vi "PicoScope6000aSetupStreaming.vi"(0 "handle in":i16=16384, 1 "Streaming Acquisition Settings":T5={"preTriggerSamples"=0, "postTriggerSamples"=1000000, "Requested sampleInterval"=1.0, "sampleIntervalTimeUnits"=3} {"sampleIntervalTimeUnits" items=["femtoseconds", "picoseconds", "nanoseconds", "microseconds", "millseconds", "seconds"]; "postTriggerSamples" format="%_6p"; "preTriggerSamples" format="%_6p"}, 2 "Buffer and Transfer Settings":T4={"startIndex"=0, "Samples"=1000000, "Down Sample Ratio"=1, "Down-Sample Mode"=2147483648} {"Down-Sample Mode" items=["None"=2147483648, "Aggregate"=1, "Decimate"=2, "Average"=4]; "Down Sample Ratio" step=1; "Samples" format="%_6p"}, 3 "enabled array":i16[](array[numeric])=[1, 1, 0, 0, 0, 0, 0, 0, 0, 0], 5 "Device Info":T1, 7 "Data Pointers In":T2, 9 "Number of Buffers":i32=1, 11 "error in (no error)":errorcluster, 12 "Auto Stop":bool) -> (4 "handle out":i16=16384, 8 "Data Pointers":T2, 13 "Actual sampleInterval":T3, 15 "error out":errorcluster)   [LabVIEW 2016]
doc: "Setup streaming Pico data buffers and first calls to ps6000aSetDataDataBuffer"
uses:
  ps6000a.dll
  shared/PicoBuffers.ctl
panel:
  in  "Dummy enabled array":i16[](array[numeric])=[1, 1, 1, 1, 1, 1, 1, 1, 1, 1]
  out "Actionflag":bool=TRUE
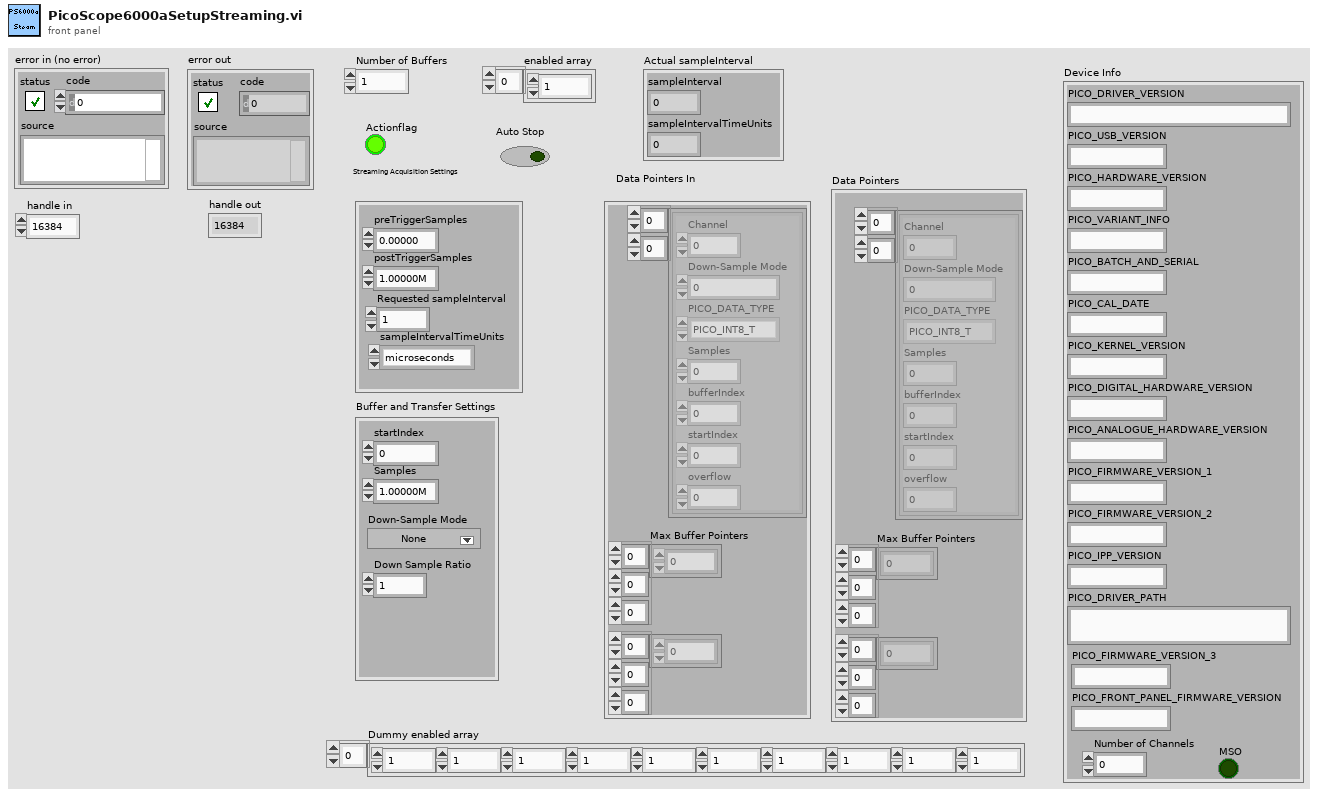
[diagram p1: front panel]
types:
  T1 = cluster{"PICO_DRIVER_VERSION":string, "PICO_USB_VERSION":string, "PICO_HARDWARE_VERSION":string, "PICO_VARIANT_INFO":string, "PICO_BATCH_AND_SERIAL":string, "PICO_CAL_DATE":string, "PICO_KERNEL_VERSION":string, "PICO_DIGITAL_HARDWARE_VERSION":string, "PICO_ANALOGUE_HARDWARE_VERSION":string, "PICO_FIRMWARE_VERSION_1":string, "PICO_FIRMWARE_VERSION_2":string, "PICO_IPP_VERSION":string, "PICO_DRIVER_PATH":string, "PICO_FIRMWARE_VERSION_3":string, "PICO_FRONT_PANEL_FIRMWARE_VERSION":string, "Number of Channels":i16, "MSO":bool}
  T2 = typedef "PicoBuffers.ctl" = cluster{"Max Buffer Pointers":u64[][][], "Min Buffer Pointers":u64[][][], "StreamingDataInfo":cluster{"Channel":u32, "Down-Sample Mode":u32, "PICO_DATA_TYPE":enum32{"PICO_INT8_T", "PICO_INT16_T", "PICO_INT32_T", "PICO_UINT32_T", "PICO_INT64_T", ""}, "Samples":i32, "bufferIndex":u64, "startIndex":i32, "overflow":i16}[][]}
  T3 = cluster{"sampleInterval":dbl, "sampleIntervalTimeUnits":u32}
  T4 = cluster{"startIndex":u64, "Samples":u64, "Down Sample Ratio":u64, "Down-Sample Mode":u32}
  T5 = cluster{"preTriggerSamples":u64, "postTriggerSamples":u64, "Requested sampleInterval":dbl, "sampleIntervalTimeUnits":u32}
  T6 = enum32{"PICO_INT8_T", "PICO_INT16_T", "PICO_INT32_T", "PICO_UINT32_T", "PICO_INT64_T", ""}
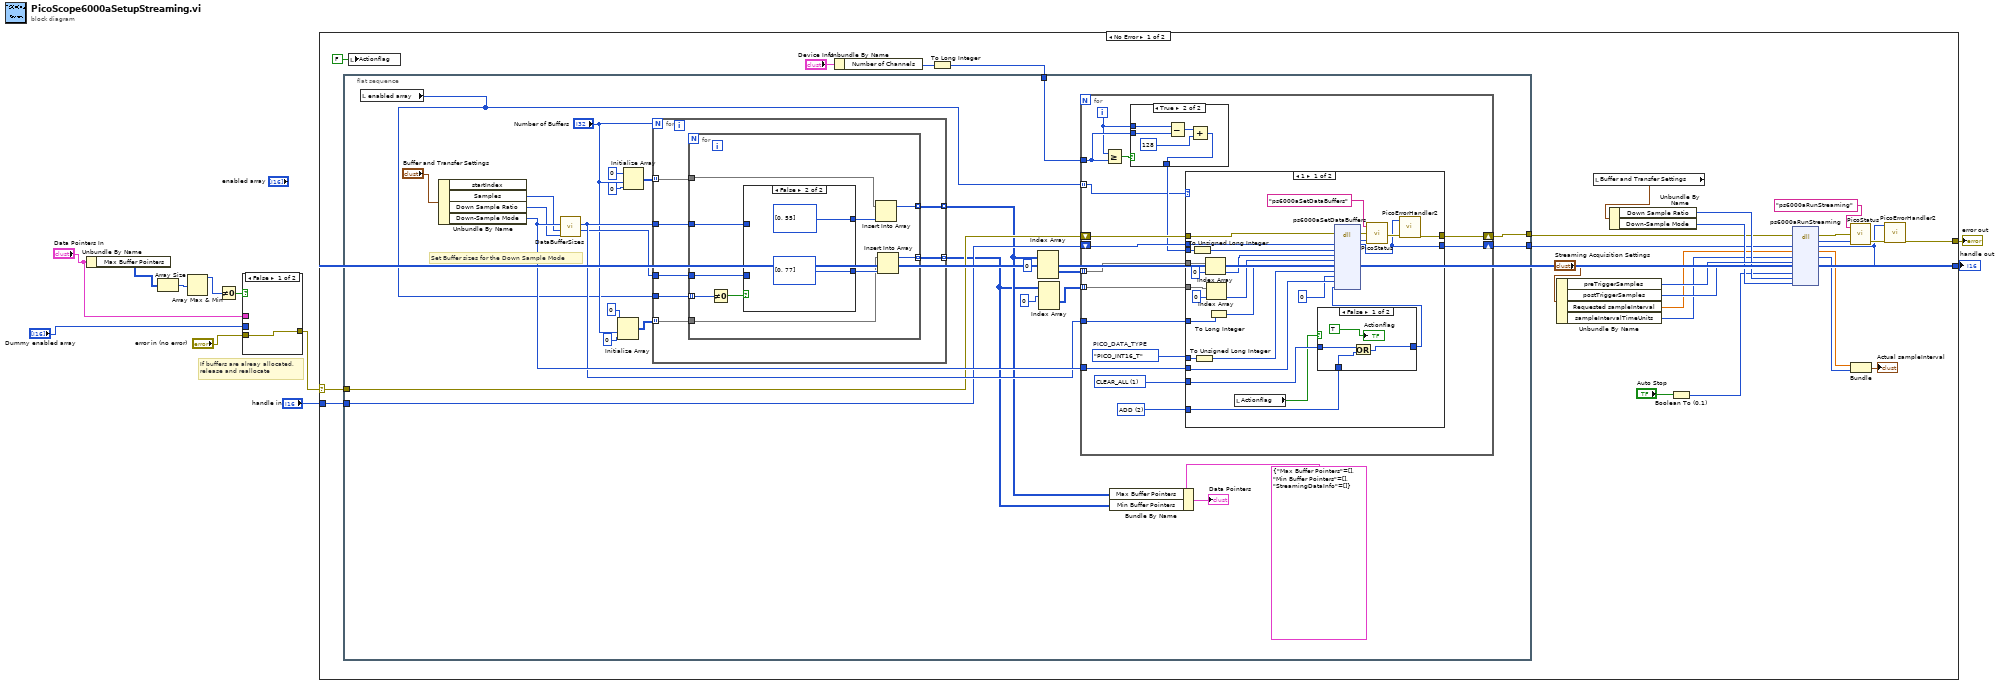
[diagram p0: block diagram]
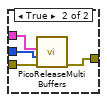
[diagram p2: hidden frame]
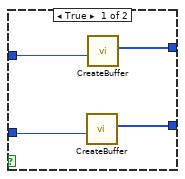
[diagram p6: hidden frame]
diagram:
  # "If buffers are alreay allocated,\nrelease and reallocate"
  n1 = Unbundle By Name("Data Pointers In") -> ("Max Buffer Pointers"=w3:u64[][][])
  n2 = Array Size(array=w3) -> (size(s)=w7:i32[])
  n3 = Array Max & Min(array=w7) -> (max value=w6:i32)  [unwired: 3 out]
  n4 = Not Equal To 0?(x=w6) -> (x != 0?=w8:bool)
  n5 = case shown="False" w8 {
    tunnel: "error in (no error)" -> [w12 w16]
    tunnel: [w12 w15] -> w4
    tunnel: "Dummy enabled array" -> [_ w14]
    tunnel: "Data Pointers In" -> [_ w13]
    frame False {
    }
    frame True {
      n6 = call "PicoReleaseMultiBuffers.vi"("error in (no error)"=w16, "Enabled array"=w14, "Data Pointers"=w13) -> ("error out"=w15:errorcluster)  [unwired: 8 in]
    }
  }
  n7 = case shown="No Error" w4 {
    selector: w4 -> [w33 w149]
    tunnel: "handle in" -> [w32 w150]
    tunnel: [w25 w150] -> w10
    tunnel: [w26 w149] -> w9
    frame No Error {
      n8 = flat-sequence {
        tunnel: w33 -> [w53]
        tunnel: w32 -> [w54]
        tunnel: [w55] -> w31
        tunnel: [w50] -> w30
        tunnel: w18 -> [w44]
        frame #0 {
          # "Set Buffer sizes for the Down Sample Mode"
          n9 = local read "enabled array"() -> (w45:i16[])
          n10 = Unbundle By Name("Buffer and Transfer Settings") -> ("Samples"=w63:u64, "Down Sample Ratio"=w62:u64, "Down-Sample Mode"=w64:u32)  [unwired: 1 out]
          n11 = call "DataBufferSizes.vi"("Down Sample Ratio"=w62, "Number of Samples"=w63, "Down-Sample Mode"=w64) -> ("min Buffer Size"=w60:i32, "Max Buffer Size"=w61:i32)  [unwired: 7 in]
          n12 = Initialize Array(u64 0 ("element"), "Number of Buffers", 0 ("dimension size")) -> (w57:u64[][])
          n13 = Initialize Array(u64 0 ("element"), "Number of Buffers", 0 ("dimension size")) -> (w65:u64[][])
          n14 = for {
            N: "Number of Buffers" -> [_]
            tunnel: w45 -> [w131]
            tunnel: w61 -> [w132]
            tunnel: w60 -> [w130]
            tunnel: [w129] -> w49 mode=indexing
            tunnel: w65 -> [w128] mode=indexing
            tunnel: w57 -> [w127] mode=indexing
            tunnel: [w126] -> w48 mode=indexing
            n15 = for {
              tunnel: w132 -> [w142]
              tunnel: w131 -> [w140] mode=indexing
              tunnel: w130 -> [w139]
              tunnel: [w137] -> w129 mode=indexing
              tunnel: w128 -> [w136]
              tunnel: w127 -> [w134]
              tunnel: [w133] -> w126 mode=indexing
              n16 = Not Equal To 0?(x=w140) -> (x != 0?=w141:bool)
              n17 = case shown="False" w141 {
                tunnel: w142 -> [w145 _]
                tunnel: w139 -> [w146 _]
                tunnel: [w144 u64[] [0, 55]] -> w138
                tunnel: [w143 u64[] [0, 77]] -> w135
                frame True {
                  n18 = call "CreateBuffer.vi"("Buffer size"=w146) -> ("Pointer and BufferSize"=w143:u64[])  [unwired: 9 in, 1 out]
                  n19 = call "CreateBuffer.vi"("Buffer size"=w145) -> ("Pointer and BufferSize"=w144:u64[])  [unwired: 9 in, 1 out]
                }
                frame False {
                }
              }
              n20 = Insert Into Array(array=w136, new element=w138) -> (w137:u64[])  [unwired: 1 in]
              n21 = Insert Into Array(array=w134, new element=w135) -> (w133:u64[])  [unwired: 1 in]
            }
          }
          n22 = Index Array(array=w49, index (dim 0)=0 ("index")) -> (element=w68:u64[][])  [unwired: 2 in]
          n23 = Index Array(array=w48, index (dim 0)=0 ("index")) -> (element=w51:u64[][])  [unwired: 2 in]
          n24 = for {
            tunnel: w64 -> [w86]
            tunnel: w61 -> [w81]
            tunnel: w45 -> [w71] mode=indexing
            tunnel: w68 -> [w80] mode=indexing
            shift-right: [w79] -> w55
            shift-left: w53 -> [w85]
            tunnel: w51 -> [w75] mode=indexing
            shift-right: [w74] -> w50
            shift-left: w54 -> [w84]
            tunnel: w44 -> [w73]
            i -> [w72]
            w76 = T6."PICO_INT16_T"  # PICO_DATA_TYPE
            w77 = u32 1 items=["NONE"=0, "CLEAR_ALL"=1, "ADD"=2, "CLEAR_THIS_DATA_BUFFER"=4096, "CLEAR_WAVEFORM_DATA_BUFFERS"=8192, "CLEAR_WAVEFORM_READ_DATA_BUFFERS"=16384] ("PicoAction 1")
            w78 = u32 2 items=["NONE"=0, "CLEAR_ALL"=1, "ADD"=2, "CLEAR_THIS_DATA_BUFFER"=4096, "CLEAR_WAVEFORM_DATA_BUFFERS"=8192, "CLEAR_WAVEFORM_READ_DATA_BUFFERS"=16384] ("PicoAction 2")
            n25 = Greater Or Equal?(x=w72, y=w73) -> (x >= y?=w83:bool)
            n26 = case shown="True" w83 {
              tunnel: [w87 w91] -> w82
              tunnel: w73 -> [_ w90]
              tunnel: w72 -> [w87 w89]
              frame False {
              }
              frame True {
                n27 = Subtract(x=w89, y=w90) -> (x-y=w88:i32)
                n28 = Add(x=w88, y=128) -> (x+y=w91:i32)
              }
            }
            n29 = case shown="1" w71 {
              tunnel: w82 -> [w107 _]
              tunnel: w85 -> [w118 w125]
              tunnel: w84 -> [w115 w124]
              tunnel: w86 -> [w112 _]
              tunnel: w76 -> [w97 _]
              tunnel: w77 -> [w102 _]
              tunnel: [w111 w125] -> w79
              tunnel: [w110 w124] -> w74
              tunnel: w81 -> [w109 _]
              tunnel: w80 -> [w103 _]
              tunnel: w78 -> [w101 _]
              tunnel: w75 -> [w93 _]
              frame 1 {
                n30 = To Unsigned Long Integer(number=w107) -> (unsigned 32bit integer=w106:u32)
                n31 = To Unsigned Long Integer(number=w97) -> (unsigned 32bit integer=w98:u32)
                n32 = Index Array(array=w103, index=0) -> (element=w104:u64)
                n33 = Index Array(array=w93, index=0) -> (element=w94:u64)
                n34 = To Long Integer(number=w109) -> (32bit integer=w108:i32)
                n35 = local read "Actionflag"() -> (w99:bool)
                n36 = case shown="False" w99 {
                  tunnel: w102 -> [w122 _]
                  tunnel: w101 -> [w121 w123]
                  tunnel: [w120 w123] -> w100
                  frame False {
                    n37 = Or(x=w122, y=w121) -> (x .or. y?=w120:u32)
                    "Actionflag" <- TRUE ("Actionflag")
                  }
                  frame True {
                  }
                }
                n38 = dll-call lib="ps6000a.dll" fn="ps6000aSetDataBuffers" ("ps3000.dll:_ps3000_open_unit@0")(error in=w118, "handle"=w115, "channel"=w106, "bufferMax"=w104, "bufferMin"=w94, "nSamples"=w108, "dataType"=w98, "waveform"=u64 0, "downSampleRatioMode"=w112, "action"=w100) -> (error out=w117:errorcluster, "PICO_STATUS"=w116:u32, "handle"=w110:i16)  [unwired: 10 in, 1 out]
                n39 = call "PicoStatus.vi"("PICO STATUS"=w116, "error in"=w117, "source"="ps6000aSetDataBuffers") -> ("error out"=w113:errorcluster)
                n40 = call "PicoErrorHandler2.vi"("error in (no error)"=w113, "handle In"=w110) -> ("error out"=w111:errorcluster)  [unwired: 9 in]
              }
              frame 0, Default {
              }
            }
          }
          n41 = Bundle By Name(cluster=T2 {"Max Buffer Pointers"=[], "Min Buffer Pointers"=[], "StreamingDataInfo"=[]} ("Data Pointers"), "Max Buffer Pointers"=w49, "Min Buffer Pointers"=w48) -> (→"Data Pointers":T2)
        }
      }
      n42 = local write "Actionflag"(FALSE ("Actionflag")) -> ()
      n43 = Unbundle By Name("Device Info") -> ("Number of Channels"=w17:i16)
      n44 = To Long Integer(number=w17) -> (32bit integer=w18:i32)
      n45 = Unbundle By Name("Streaming Acquisition Settings") -> ("preTriggerSamples"=w38:u64, "postTriggerSamples"=w37:u64, "Requested sampleInterval"=w29:dbl, "sampleIntervalTimeUnits"=w28:u32)
      n46 = local read "Buffer and Transfer Settings"() -> (w36:T4)
      n47 = Unbundle By Name(w36) -> ("Down Sample Ratio"=w35:u64, "Down-Sample Mode"=w34:u32)
      n48 = Boolean To (0,1)(Boolean="Auto Stop") -> (0, 1=w20:i16)
      n49 = dll-call lib="ps6000a.dll" fn="ps6000aRunStreaming" ("ps3000.dll:_ps3000_open_unit@0")(error in=w31, "handle"=w30, "sampleInterval"=w29, "sampleIntervalTimeUnits"=w28, "maxPreTriggerSamples"=w38, "maxPostPreTriggerSamples"=w37, "autoStop"=w20, "downSampleRatio"=w35, "downSampleRatioMode"=w34) -> (error out=w42:errorcluster, "PICO_STATUS"=w41:u32, "handle"=w25:i16, "sampleInterval"=w24:dbl, "sampleIntervalTimeUnits"=w23:u32)  [unwired: 7 in, 1 out]
      n50 = call "PicoStatus.vi"("PICO STATUS"=w41, "error in"=w42, "source"="ps6000aRunStreaming") -> ("error out"=w43:errorcluster)
      n51 = Bundle("sampleInterval"=w24, "sampleIntervalTimeUnits"=w23) -> (→"Actual sampleInterval":T3)  [unwired: 1 in]
      n52 = call "PicoErrorHandler2.vi"("error in (no error)"=w43, "handle In"=w25) -> ("error out"=w26:errorcluster)  [unwired: 9 in]
    }
    frame Error {
    }
  }
  "handle out" <- w10
  "error out" <- w9
